vi "All VIs.vi"   [LabVIEW 2027]
uses:
  <vilib>/REVLibDriver/REVLibDriver.lvlib
  <resource>/objmgr/REVSpark.rc
  <vilib>/MRC/MrcLib.lvlib
  <vilib>/MRC/MrcLib/VIs/IMU/IMU Get Yaw Flat.vi
  <vilib>/MRC/MrcLib/VIs/IMU/IMU Get Euler Angle Flat.vi
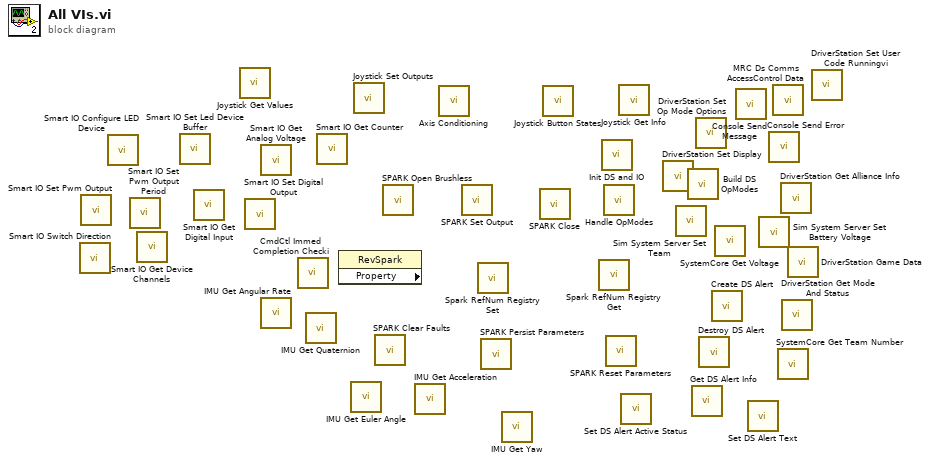
[diagram p0: block diagram]
diagram:
  n1 = call <vilib>:"Smart IO Switch Direction.vi"() -> ()  [unwired: 11 in, 1 out]
  n2 = call <vilib>:"Smart IO Set Pwm Output.vi"() -> ()  [unwired: 11 in, 1 out]
  n3 = call <vilib>:"Smart IO Configure LED Device.vi"() -> ()  [unwired: 10 in, 2 out]
  n4 = call <vilib>:"Smart IO Set Pwm Output Period.vi"() -> ()  [unwired: 11 in, 1 out]
  n5 = call <vilib>:"Smart IO Get Device Channels.vi"() -> ()  [unwired: 10 in, 2 out]
  n6 = call <vilib>:"Smart IO Set Led Device Buffer.vi"() -> ()  [unwired: 11 in, 1 out]
  n7 = call <vilib>:"Smart IO Get Digital Input.vi"() -> ()  [unwired: 10 in, 2 out]
  n8 = call <vilib>:"Joystick Get Values.vi"() -> ()  [unwired: 6 in, 6 out]
  n9 = call <vilib>:"Smart IO Set Digital Output.vi"() -> ()  [unwired: 11 in, 1 out]
  n10 = call <vilib>:"Smart IO Get Analog Voltage.vi"() -> ()  [unwired: 9 in, 3 out]
  n11 = call <vilib>:"IMU Get Angular Rate.vi"() -> ()  [unwired: 9 in, 3 out]
  n12 = call <vilib>:"CmdCtl Immed Completion Checki.vi"() -> ()  [unwired: 11 in, 1 out]
  n13 = call <vilib>:"IMU Get Quaternion.vi"() -> ()  [unwired: 9 in, 3 out]
  n14 = call <vilib>:"Smart IO Get Counter.vi"() -> ()  [unwired: 10 in, 2 out]
  n15 = property class="RevSpark" props=[]() -> ()  [unwired: 2 in, 3 out]
  n16 = call-poly <vilib>:"IMU Get Euler Angle.vi"() -> ()  [unwired: 9 in, 3 out]
  n17 = call <vilib>:"Joystick Set Outputs.vi"() -> ()  [unwired: 10 in, 2 out]
  n18 = call <vilib>:"SPARK Clear Faults.vi"() -> ()  [unwired: 10 in, 2 out]
  n19 = call <vilib>:"SPARK Open Brushless.vi"() -> ()  [unwired: 10 in, 2 out]
  n20 = call <vilib>:"IMU Get Acceleration.vi"() -> ()  [unwired: 9 in, 3 out]
  n21 = call <vilib>:"Axis Conditioning.vi"() -> ()  [unwired: 10 in, 2 out]
  n22 = call <vilib>:"SPARK Set Output.vi"() -> ()  [unwired: 10 in, 2 out]
  n23 = call <vilib>:"Spark RefNum Registry Set.vi"() -> ()  [unwired: 10 in, 2 out]
  n24 = call <vilib>:"SPARK Persist Parameters.vi"() -> ()  [unwired: 10 in, 2 out]
  n25 = call-poly <vilib>:"IMU Get Yaw.vi"() -> ()  [unwired: 9 in, 3 out]
  n26 = call <vilib>:"SPARK Close.vi"() -> ()  [unwired: 11 in, 1 out]
  n27 = call <vilib>:"Joystick Button States.vi"() -> ()  [unwired: 8 in, 4 out]
  n28 = call <vilib>:"Spark RefNum Registry Get.vi"() -> ()  [unwired: 10 in, 2 out]
  n29 = call <vilib>:"Init DS and IO.vi"() -> ()  [unwired: 10 in, 2 out]
  n30 = call <vilib>:"Handle OpModes.vi"() -> ()  [unwired: 12 in]
  n31 = call <vilib>:"SPARK Reset Parameters.vi"() -> ()  [unwired: 10 in, 2 out]
  n32 = call <vilib>:"Joystick Get Info.vi"() -> ()  [unwired: 9 in, 3 out]
  n33 = call <vilib>:"Set DS Alert Active Status.vi"() -> ()  [unwired: 11 in, 1 out]
  n34 = call <vilib>:"DriverStation Set Display.vi"() -> ()  [unwired: 11 in, 1 out]
  n35 = call <vilib>:"Sim System Server Set Team.vi"() -> ()  [unwired: 11 in, 1 out]
  n36 = call <vilib>:"Build DS OpModes.vi"() -> ()  [unwired: 11 in, 1 out]
  n37 = call <vilib>:"Get DS Alert Info.vi"() -> ()  [unwired: 11 in, 1 out]
  n38 = call <vilib>:"DriverStation Set Op Mode Options.vi"() -> ()  [unwired: 11 in, 1 out]
  n39 = call <vilib>:"Destroy DS Alert.vi"() -> ()  [unwired: 11 in, 1 out]
  n40 = call <vilib>:"Create DS Alert.vi"() -> ()  [unwired: 10 in, 2 out]
  n41 = call <vilib>:"SystemCore Get Voltage.vi"() -> ()  [unwired: 14 in, 2 out]
  n42 = call <vilib>:"Console Send Message.vi"() -> ()  [unwired: 15 in, 1 out]
  n43 = call <vilib>:"Set DS Alert Text.vi"() -> ()  [unwired: 11 in, 1 out]
  n44 = call <vilib>:"Sim System Server Set Battery Voltage.vi"() -> ()  [unwired: 11 in, 1 out]
  n45 = call <vilib>:"Console Send Error.vi"() -> ()  [unwired: 15 in, 1 out]
  n46 = call <vilib>:"MRC Ds Comms AccessControl Data.vi"() -> ()  [unwired: 8 in, 4 out]
  n47 = call <vilib>:"SystemCore Get Team Number.vi"() -> ()  [unwired: 14 in, 2 out]
  n48 = call <vilib>:"DriverStation Get Alliance Info.vi"() -> ()  [unwired: 7 in, 5 out]
  n49 = call <vilib>:"DriverStation Get Mode And Status.vi"() -> ()  [unwired: 6 in, 6 out]
  n50 = call <vilib>:"DriverStation Game Data.vi"() -> ()  [unwired: 11 in, 1 out]
  n51 = call <vilib>:"DriverStation Set User Code Runningvi.vi"() -> ()  [unwired: 11 in, 1 out]
